vi "Read Numeric Inputs.vi"(8 "error in (no error)":errorcluster, 11 "Modbus in":refnum<class "Modbus.lvclass">) -> (0 "error out":errorcluster, 3 "Modbus out":refnum<class "Modbus.lvclass">)   [LabVIEW 2026, in "Modbus.lvlib" / "Modbus.lvclass"]
uses:
  Modbus.lvclass
  C:/Program Files/National Instruments/LabVIEW 2026/vi.lib/FlexLogger/SDK/PluginSDK.lvlibp/PEFClasses/SDK/Plugin/Plugin.lvclass
  Modbus.lvclass/Modbus.ctl
  <vilib>/FlexLogger/SDK/PluginSDK.lvlibp/PEFClasses/SDK/Plugin/DataHelpers/Write 1D DBL (NChan 1Sample).vi
  C:/Program Files/National Instruments/LabVIEW 2026/vi.lib/FlexLogger/SDK/PluginSDK.lvlibp/PEFClasses/SDK/Processing Element/Processing Element.lvclass
  D:/Work/FlexLogger/Features/Modbus Plugin/Modbus - Working Copy/Modbus/Modbus.lvclass
  <vilib>/FlexLogger/SDK/PluginSDK.lvlibp/PEFClasses/SDK/Plugin/Plugin.lvclass
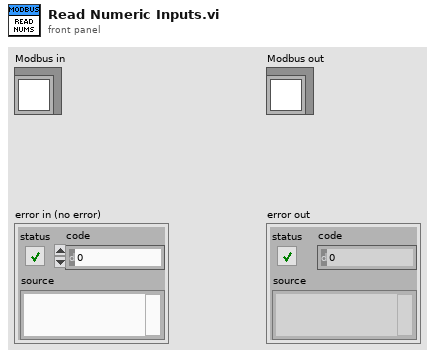
[diagram p1: front panel]
types:
  T1 = typedef "Modbus.lvlib/Modbus.lvclass/Numeric Data.ctl" = cluster{"Channel UID":string, "Valid?":bool, "Table":T2, "Address":i32, "Quantity":u16, "Size":T3, "Data Type":T4, "Location":T5}
  T2 = typedef "Modbus.lvlib/Modbus.lvclass/Modbus Table.ctl" = enum16{"Discrete Inputs", "Coils", "Input Registers", "Holding Registers"}
  T3 = typedef "Modbus.lvlib/Modbus.lvclass/Numeric Size.ctl" = enum16{"8-bit (Half register)", "16-bit (One register)", "32-bit (Two registers)", "64-bit (Four registers)"}
  T4 = typedef "Modbus.lvlib/Modbus.lvclass/Numeric Data Type.ctl" = enum16{"Unsigned Integer", "Signed Integer", "Floating Point"}
  T5 = typedef "Modbus.lvlib/Modbus.lvclass/Numeric Location.ctl" = enum16{"Low Byte", "High Byte"}
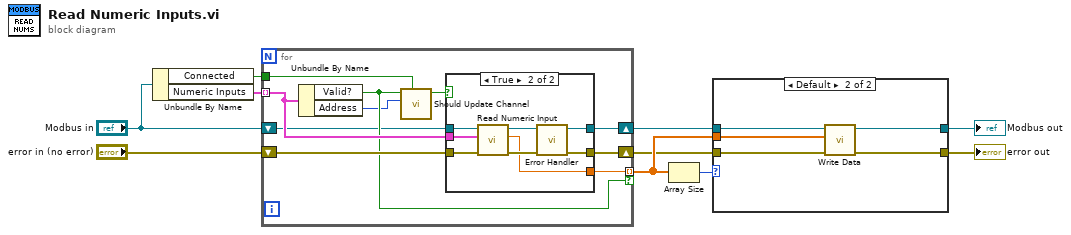
[diagram p0: block diagram]
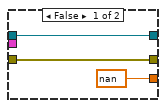
[diagram p2: hidden frame]
diagram:
  n1 = Unbundle By Name("Modbus in") -> ("Connected"=w6:bool, "Numeric Inputs"=w2:T1[])
  n2 = for {
    tunnel: w2 -> [w18] mode=indexing
    tunnel: [w19] -> w9 mode=indexing if=w15
    shift-right: [w20] -> w8
    shift-left: "error in (no error)" -> [w16]
    tunnel: w6 -> [w14]
    shift-right: [w12] -> w5
    shift-left: "Modbus in" -> [w13]
    n3 = Unbundle By Name(w18) -> ("Valid?"=w15:bool, "Address"=w11:i32)
    n4 = call "Should Update Channel.vi"("Connected?"=w14, "Address"=w11, "Valid?"=w15) -> ("Update?"=w17:bool)  [unwired: 8 in]
    n5 = case shown="True" w17 {
      tunnel: [w23 w31] -> w20
      tunnel: [nan w24] -> w19
      tunnel: w18 -> [_ w29]
      tunnel: w16 -> [w23 w28]
      tunnel: w13 -> [w21 w27]
      tunnel: [w21 w30] -> w12
      frame False {
      }
      frame True {
        n6 = call "Read Numeric Input.vi"("error in (no error)"=w28, "Numeric Input in"=w29, "Modbus in"=w27) -> ("error out"=w25:errorcluster, "Numeric Value"=w24:dbl, "Modbus out"=w26:refnum<class "Modbus.lvclass">)  [unwired: 6 in]
        n7 = call "Error Handler.vi"("error in (no error)"=w25, "Modbus in"=w26) -> ("error out"=w31:errorcluster, "Modbus out"=w30:refnum<class "Modbus.lvclass">)  [unwired: 8 in]
      }
    }
  }
  n8 = Array Size(array=w9) -> (size(s)=w4:i32)
  n9 = case shown="Default" w4 {
    tunnel: w5 -> [w32 w38]
    tunnel: w9 -> [_ w37]
    tunnel: w8 -> [w33 w36]
    tunnel: [w32 w35] -> w10
    tunnel: [w33 w34] -> w7
    frame 0 {
    }
    frame Default {
      n10 = call-poly <vilib>:"Write Data.vi"("error in (no error)"=w36, "Data"=w37, "Plugin in"=w38) -> ("error out"=w34:errorcluster, "Plugin out"=w35:refnum<class "Modbus.lvclass">)  [unwired: 7 in]
    }
  }
  "Modbus out" <- w10
  "error out" <- w7
